vi "Module Loop.vi"(8 "error in (no error)":errorcluster, 11 "DAQmxDO in":refnum<class "DAQmxDO.lvclass">) -> (0 "error out":errorcluster, 3 "DAQmxDO out":refnum<class "DAQmxDO.lvclass">)   [LabVIEW 2020, in "VolatusDAQ.lvlib" / "DAQmxDO.lvclass"]
uses:
  DAQmxDO.lvclass
  C:/dev/lv20CE/relink/lv-volatus/Volatus/Module/Module.lvclass
  DAQmxDO.lvclass/DAQmxDO.ctl
  Volatus/Module/Module.lvclass
  Volatus/MessageQ/MessageQ.lvclass/MessageQ.ctl
  messages/CmdDigital/Class/Msg.lvclass
  C:/dev/lv20CE/relink/lv-protoc/LV-Proto/Message/Message.lvclass
  messages/CmdDigital/Class/Msg.lvclass/Msg.ctl
  Volatus/Module/Module.lvclass/Module.ctl
  messages/CmdDigital/Data.ctl
  VolatusData/Scaling/Scaling.lvclass/Scaling.ctl
  messages/CmdDigitalMultiple/Class/Msg.lvclass
  messages/CmdDigitalMultiple/Class/Msg.lvclass/Msg.ctl
  messages/CmdDigitalMultiple/Data.ctl
  <vilib>/DAQmx/write.llb/DAQmx Write (Digital 1D Bool NChan 1Samp 1Line).vi
  VolatusData/Send New Data (Array).vi
  Volatus/Module/Self Q.vi
  Volatus/MessageQ/Send.vi
  VolatusData/Scaling/Scale Channel (Scalar).vi
  Volatus/Module/Report Event.vi
  lv-vecto/Vecto/Bool to String.vi
  Volatus/Module/Format Bool Array Cmd.vi
  VolatusData/Scaling/Polynomial Evaluate.vi
  VolatusData/Scaling/Expo Scale Value.vi
  <vilib>/AdvancedString/1D String Array to Delimited String.vi
  VolatusData/Scaling/Polynomial Remove Trailing Zeros.vi
  lv-vecto/Vecto/Group DBL/Group DBL.lvclass
  C:/dev/lv20CE/relink/lv-vecto/Vecto/Group/Group.lvclass
  <vilib>/DAQmx/miscellaneous.llb/DAQmx Fill In Error Info.vi
  Volatus/VolatusAPI/Report Event.vi
  <vilib>/Utility/error.llb/Error Cluster From Error Code.vi
  VolatusData/Scaling/Scaling.lvclass
  lv-vecto/Vecto/Group/Group.lvclass
  lv-vecto/Vecto/Vecto.lvlib
  messages/CmdDigital/CmdDigital.lvlib
  messages/CmdDigitalMultiple/CmdDigitalMultiple.lvlib
  C:/dev/lv20CE/relink/lv-volatus/VolatusDAQ/DAQmxDO/DAQmxDO.lvclass
  C:/dev/lv20CE/relink/lv-vecto/Vecto/Group DBL/Group DBL.lvclass
  C:/dev/lv20CE/relink/lv-volatus/messages/CmdDigital/Class/Msg.lvclass
  C:/dev/lv20CE/relink/lv-volatus/messages/CmdDigitalMultiple/Class/Msg.lvclass
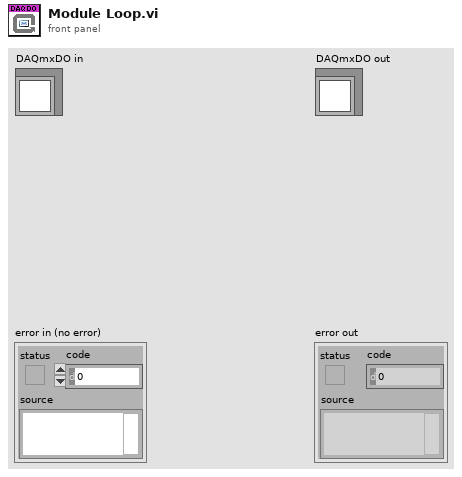
[diagram p1: front panel]
types:
  T1 = enum32{"Invalid", "Standard", "Closed", "Hidden", "Minimized", "Maximized"}
  T2 = typedef "CmdDigital.lvlib/Data.ctl" = cluster{"channel":string, "value":bool}
  T3 = typedef "CmdDigitalMultiple.lvlib/Data.ctl" = cluster{"values":T2[]}
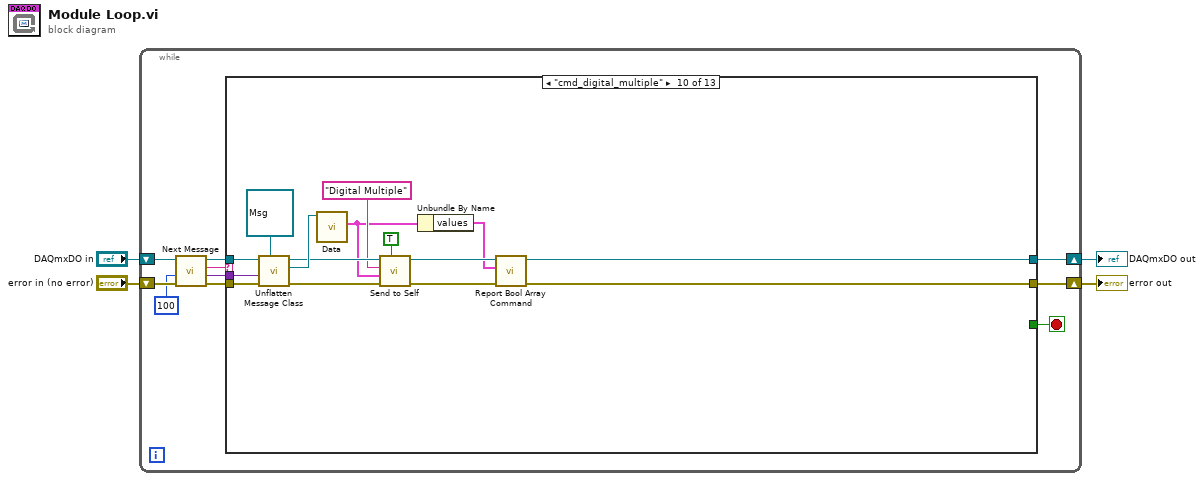
[diagram p0: block diagram]
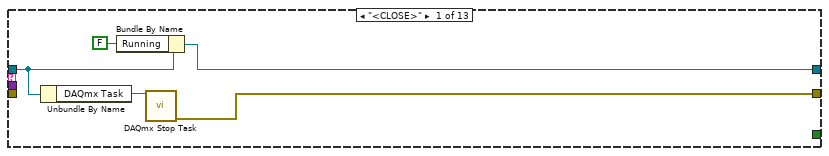
[diagram p2: hidden frame]
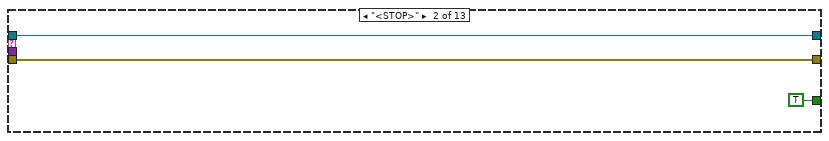
[diagram p3: hidden frame]
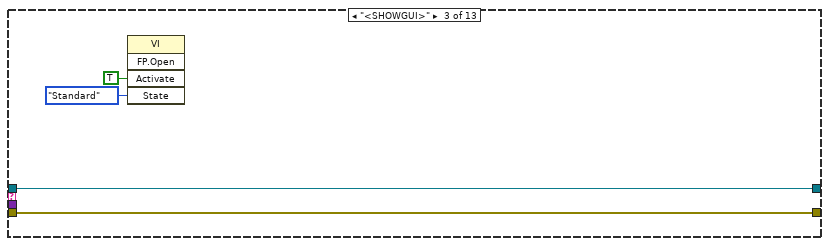
[diagram p4: hidden frame]
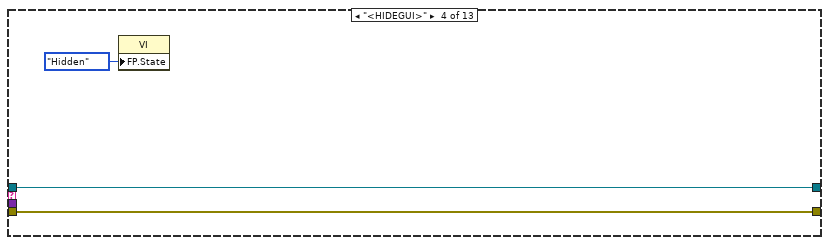
[diagram p5: hidden frame]
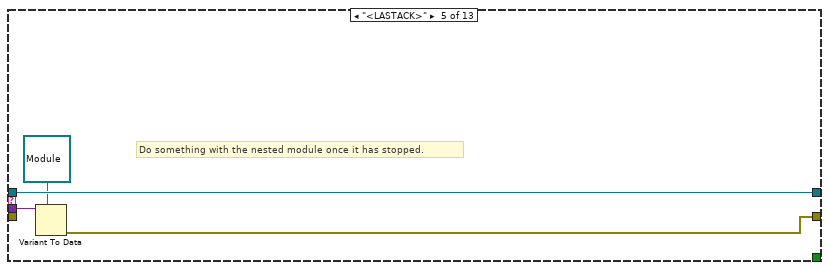
[diagram p6: hidden frame]
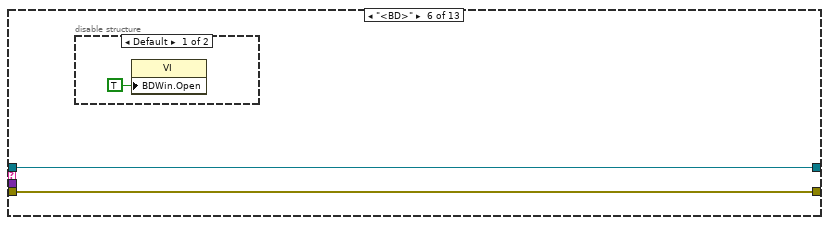
[diagram p7: hidden frame]
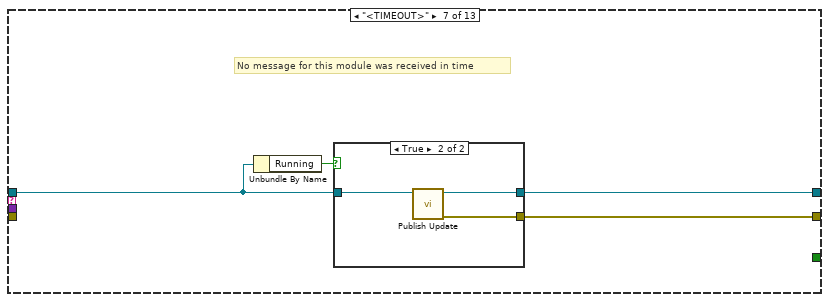
[diagram p9: hidden frame]
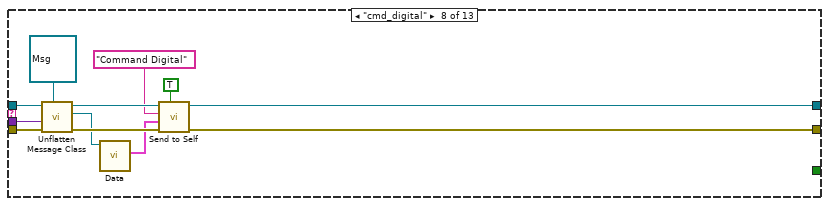
[diagram p11: hidden frame]
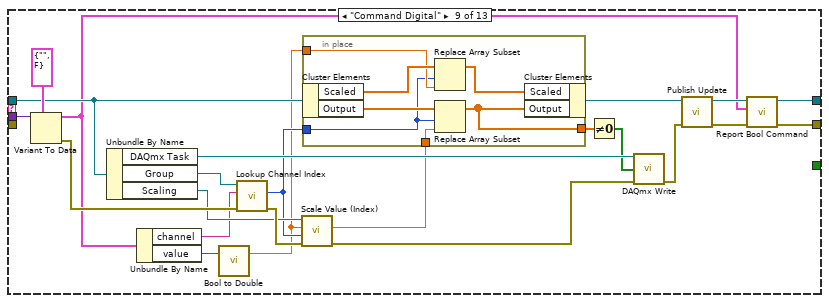
[diagram p12: hidden frame]
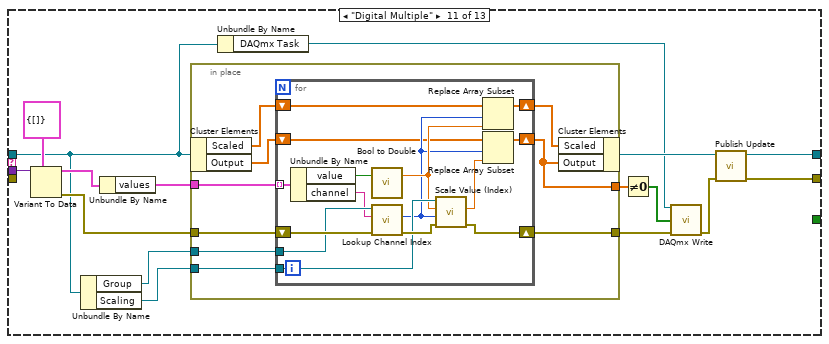
[diagram p13: hidden frame]
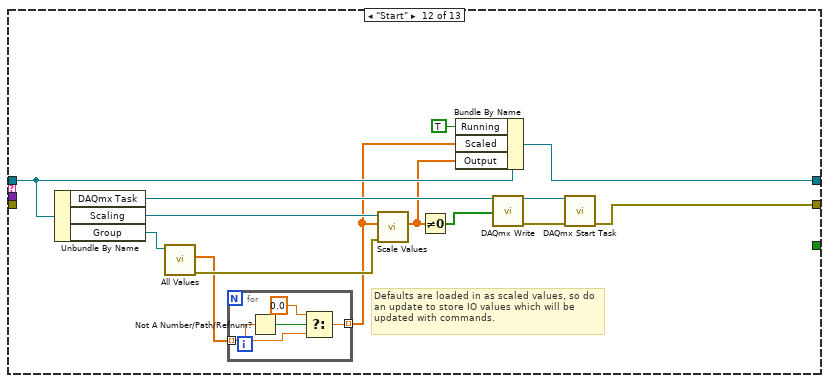
[diagram p14: hidden frame]
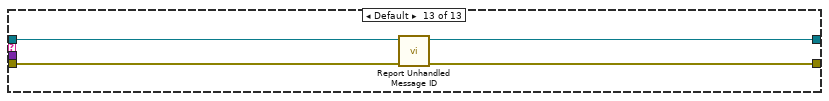
[diagram p15: hidden frame]
diagram:
  n1 = while {
    shift-right: [w9] -> w2
    shift-left: "DAQmxDO in" -> [w14]
    shift-right: [w8] -> w1
    shift-left: "error in (no error)" -> [w13]
    stop <- w7 stop-if-true
    n2 = call "Next Message.vi"("error in (no error)"=w13, "Timeout ms (-1)"=100, "Module in"=w14) -> ("error out"=w12:errorcluster, "Data"=w6:variant, "ID"=w11:string, "Module out"=w10:refnum<class "DAQmxDO.lvclass">)  [unwired: 5 in]
    n3 = case shown="\"cmd_digital_multiple\"" w11 {
      tunnel: w12 -> [_ w21 w25 w28 _ w34 _ w54 _ w98 _ _ w163]
      tunnel: w10 -> [w18 w22 w26 w29 w33 w35 w38 w55 w70 w99 w106 w149 w161]
      tunnel: [w16 w22 w26 w29 w33 w35 w39 w46 w58 w89 w102 w145 w160] -> w9
      tunnel: [w17 w21 w25 w28 w30 w34 w40 w47 w60 w91 w103 w148 w162] -> w8
      tunnel: [_ TRUE _ _ _ _ _ _ _ _ _ _ _] -> w7
      tunnel: w6 -> [_ _ _ _ w32 _ _ w53 w73 w97 w114 _ _]
      frame "<CLOSE>" {
        n4 = Unbundle By Name(w18) -> ("DAQmx Task"=w19:refnum<k21>)
        n5 = Bundle By Name(cluster=w18, "Running"=FALSE) -> (w16:refnum<class "DAQmxDO.lvclass">)
        n6 = call <vilib>:"DAQmx Stop Task.vi"("task/channels in"=w19) -> ("error out"=w17:errorcluster)  [unwired: 13 in, 1 out]
      }
      frame "<STOP>" {
      }
      frame "<SHOWGUI>" {
        n7 = invoke class="VI" method="FP.Open"("Activate"=TRUE ("Activate?"), "State"=T1."Standard") -> ()  [unwired: 3 in, 5 out]
      }
      frame "<HIDEGUI>" {
        n8 = property class="VI"("FP.State"=T1."Hidden" ("Front Panel Window:State")) -> ()  [unwired: 2 in, 2 out]
      }
      frame "<LASTACK>" {
        # "Do something with the nested module once it has stopped."
        n9 = Variant To Data(type=refnum<class "Module.lvclass"> refnum ("Volatus:Module"), Variant=w32) -> (error out=w30:errorcluster)  [unwired: 1 in, 1 out]
      }
      frame "<BD>" {
        n10 = disable-structure shown="Default" {
          frame condition #0 (active) {
            n11 = property class="VI"("BDWin.Open"=TRUE ("Block Diagram Window:Open")) -> ()  [unwired: 2 in, 2 out]
          }
          frame condition #1 {
          }
        }
      }
      frame "<TIMEOUT>" {
        # "No message for this module was received in time"
        n12 = Unbundle By Name(w38) -> ("Running"=w37:bool)
        n13 = case shown="True" w37 {
          tunnel: [_ w42] -> w40
          tunnel: [w41 w43] -> w39
          tunnel: w38 -> [w41 w44]
          frame False {
          }
          frame True {
            n14 = call "Publish Update.vi"("DAQmxDO in"=w44) -> ("error out"=w42:errorcluster, "DAQmxDO out"=w43:refnum<class "DAQmxDO.lvclass">)  [unwired: 9 in]
          }
        }
      }
      frame "cmd_digital" {
        n15 = call "Unflatten Message Class.vi"("Message Type"=refnum<class "Msg.lvclass"> refnum ("CmdDigital.lvlib:Msg.lvclass"), "error in (no error)"=w54, "Data"=w53, "Module in"=w55) -> ("error out"=w51:errorcluster, "Message"=w45:refnum<class "Msg.lvclass">, "Module out"=w52:refnum<class "DAQmxDO.lvclass">)  [unwired: 4 in, 1 out]
        n16 = call "Data.vi"("PB Msg Template in"=w45) -> ("Data"=w48:T2)  [unwired: 8 in, 2 out]
        n17 = call "Send to Self.vi"("High Priority (F)"=TRUE, "error in (no error)"=w51, "Data"=w48, "Message ID"="Command Digital", "Module in"=w52) -> ("error out"=w47:errorcluster, "Module out"=w46:refnum<class "DAQmxDO.lvclass">)  [unwired: 5 in]
      }
      frame "Command Digital" {
        n18 = Variant To Data(type=T2 {"channel"="", "value"=FALSE} ("Data"), Variant=w73) -> (data=w57:T2, error out=w79:errorcluster)  [unwired: 1 in]
        n19 = Unbundle By Name(w70) -> ("DAQmx Task"=w74:refnum<k21>, "Group"=w77:refnum<class "Group DBL.lvclass">, "Scaling"=w76:refnum<class "Scaling.lvclass">)
        n20 = Unbundle By Name(w57) -> ("channel"=w71:string, "value"=w75:bool)
        n21 = call "Bool to Double.vi"("Bool"=w75) -> ("Double"=w68:dbl)  [unwired: 2 in]
        n22 = call "Lookup Channel Index.vi"("error in (no error)"=w79, "Channel Name"=w71, "Group in"=w77) -> ("error out"=w78:errorcluster, "Index"=w69:i32)  [unwired: 6 in, 1 out]
        n23 = call "Scale Value (Index).vi"("error in (no error)"=w78, "Index"=w69, "Value"=w68, "VolatusScaling in"=w76) -> ("error out"=w64:errorcluster, "Scaled Value"=w67:dbl)  [unwired: 5 in, 1 out]
        n24 = in-place {
          in-place-border: w69 -> [w82]
          in-place-border: w68 -> [w85]
          in-place-border: w67 -> [w81]
          in-place-border: [w80] -> w66
          n25 = in-place-cluster #1(w70) -> ("Scaled"=w86:dbl[], "Output"=w83:dbl[])
          n26 = Replace Array Subset(array=w86, new element=w85, index=w82) -> (w84:dbl[])
          n27 = Replace Array Subset(array=w83, new element=w81, index=w82) -> (w80:dbl[])
          n28 = in-place-cluster #1("Scaled"=w84, "Output"=w80) -> (w63:refnum<class "DAQmxDO.lvclass">)
        }
        n29 = Not Equal To 0?(x=w66) -> (x != 0?=w65:bool[])
        n30 = call-poly <vilib>:"DAQmx Write.vi"("task/channels in"=w74, "data"=w65, "error in"=w64) -> ("error out"=w62:errorcluster)  [unwired: 10 in, 2 out]
        n31 = call "Publish Update.vi"("error in (no error)"=w62, "DAQmxDO in"=w63) -> ("error out"=w61:errorcluster, "DAQmxDO out"=w59:refnum<class "DAQmxDO.lvclass">)  [unwired: 8 in]
        n32 = call "Report Bool Command.vi"("error in (no error)"=w61, "Command"=w57, "Module in"=w59) -> ("error out"=w60:errorcluster, "Module out"=w58:refnum<class "DAQmxDO.lvclass">)  [unwired: 7 in]
      }
      frame "cmd_digital_multiple" {
        n33 = call "Unflatten Message Class.vi"("Message Type"=refnum<class "Msg.lvclass"> refnum ("CmdDigitalMultiple.lvlib:Msg.lvclass"), "error in (no error)"=w98, "Data"=w97, "Module in"=w99) -> ("error out"=w95:errorcluster, "Message"=w100:refnum<class "Msg.lvclass">, "Module out"=w96:refnum<class "DAQmxDO.lvclass">)  [unwired: 4 in, 1 out]
        n34 = call "Data.vi"("PB Msg Template in"=w100) -> ("Data"=w88:T3)  [unwired: 8 in, 2 out]
        n35 = call "Send to Self.vi"("High Priority (F)"=TRUE, "error in (no error)"=w95, "Data"=w88, "Message ID"="Digital Multiple", "Module in"=w96) -> ("error out"=w92:errorcluster, "Module out"=w90:refnum<class "DAQmxDO.lvclass">)  [unwired: 5 in]
        n36 = Unbundle By Name(w88) -> ("values"=w87:T2[])
        n37 = call "Report Bool Array Command.vi"("error in (no error)"=w92, "Command"=w87, "Module in"=w90) -> ("error out"=w91:errorcluster, "Module out"=w89:refnum<class "DAQmxDO.lvclass">)  [unwired: 7 in]
      }
      frame "Digital Multiple" {
        n38 = Variant To Data(type=T3 {"values"=[]} ("input cluster"), Variant=w114) -> (data=w112:T3, error out=w111:errorcluster)  [unwired: 1 in]
        n39 = Unbundle By Name(w106) -> ("Group"=w116:refnum<class "Group DBL.lvclass">, "Scaling"=w115:refnum<class "Scaling.lvclass">)
        n40 = Unbundle By Name(w112) -> ("values"=w104:T2[])
        n41 = in-place {
          in-place-border: [w126] -> w117
          in-place-border: w116 -> [w125]
          in-place-border: w115 -> [w124]
          in-place-border: w104 -> [w123]
          in-place-border: w111 -> [w122]
          in-place-border: [w118] -> w109
          n42 = in-place-cluster #2(w106) -> ("Scaled"=w121:dbl[], "Output"=w120:dbl[])
          n43 = for {
            tunnel: w124 -> [w138]
            shift-right: [w134] -> w126
            shift-left: w122 -> [w140]
            tunnel: w123 -> [w137] mode=indexing
            tunnel: w125 -> [w139]
            shift-right: [w130] -> w118
            shift-left: w120 -> [w128]
            shift-right: [w129] -> w119
            shift-left: w121 -> [w127]
            n44 = Unbundle By Name(w137) -> ("value"=w136:bool, "channel"=w135:string)
            n45 = call "Bool to Double.vi"("Bool"=w136) -> ("Double"=w133:dbl)  [unwired: 2 in]
            n46 = call "Lookup Channel Index.vi"("error in (no error)"=w140, "Channel Name"=w135, "Group in"=w139) -> ("error out"=w141:errorcluster, "Index"=w131:i32)  [unwired: 6 in, 1 out]
            n47 = call "Scale Value (Index).vi"("error in (no error)"=w141, "Index"=w131, "Value"=w133, "VolatusScaling in"=w138) -> ("error out"=w134:errorcluster, "Scaled Value"=w132:dbl)  [unwired: 5 in, 1 out]
            n48 = Replace Array Subset(array=w127, new element=w133, index=w131) -> (w129:dbl[])
            n49 = Replace Array Subset(array=w128, new element=w132, index=w131) -> (w130:dbl[])
          }
          n50 = in-place-cluster #2("Scaled"=w119, "Output"=w118) -> (w110:refnum<class "DAQmxDO.lvclass">)
        }
        n51 = Unbundle By Name(w106) -> ("DAQmx Task"=w105:refnum<k21>)
        n52 = Not Equal To 0?(x=w109) -> (x != 0?=w108:bool[])
        n53 = call-poly <vilib>:"DAQmx Write.vi"("task/channels in"=w105, "data"=w108, "error in"=w117) -> ("error out"=w107:errorcluster)  [unwired: 10 in, 2 out]
        n54 = call "Publish Update.vi"("error in (no error)"=w107, "DAQmxDO in"=w110) -> ("error out"=w103:errorcluster, "DAQmxDO out"=w102:refnum<class "DAQmxDO.lvclass">)  [unwired: 8 in]
      }
      frame "Start" {
        # "Defaults are loaded in as scaled values, so do an update to store IO values which will be updated with commands."
        n55 = Unbundle By Name(w149) -> ("DAQmx Task"=w152:refnum<k21>, "Scaling"=w153:refnum<class "Scaling.lvclass">, "Group"=w154:refnum<class "Group DBL.lvclass">)
        n56 = call "All Values.vi"("Group in"=w154) -> ("error out"=w155:errorcluster, "Scaled"=w146:dbl[])  [unwired: 6 in, 3 out]
        n57 = for {
          tunnel: w146 -> [w158] mode=indexing
          tunnel: [w156] -> w144 mode=indexing
          n58 = Not A Number/Path/Refnum?(number/path/refnum=w158) -> (NaN/Path/Refnum?=w159:bool)
          n59 = Select(t=0.0, s=w159, f=w158) -> (s? t:f=w156:dbl)
        }
        n60 = call "Scale Values.vi"("error in (no error)"=w155, "Values"=w144, "VolatusScaling in"=w153) -> ("Scaled Values"=w143:dbl[])  [unwired: 6 in, 2 out]
        n61 = Not Equal To 0?(x=w143) -> (x != 0?=w147:bool[])
        n62 = Bundle By Name(cluster=w149, "Running"=TRUE, "Scaled"=w144, "Output"=w143) -> (w145:refnum<class "DAQmxDO.lvclass">)
        n63 = call-poly <vilib>:"DAQmx Write.vi"("task/channels in"=w152, "data"=w147) -> ("task out"=w151:refnum<k21>, "error out"=w150:errorcluster)  [unwired: 11 in, 1 out]
        n64 = call <vilib>:"DAQmx Start Task.vi"("task/channels in"=w151, "error in"=w150) -> ("error out"=w148:errorcluster)  [unwired: 12 in, 1 out]
      }
      frame Default {
        n65 = call "Report Unhandled Message ID.vi"("error in (no error)"=w163, "Module in"=w161) -> ("error out"=w162:errorcluster, "Module out"=w160:refnum<class "DAQmxDO.lvclass">)  [unwired: 8 in]
      }
    }
  }
  "error out" <- w1
  "DAQmxDO out" <- w2
